vi "Plugin_Collect_Result.vi"(8 "error in (no error)":errorcluster={"status"=FALSE, "code"=0, "source"="\"\""}, 10 "output data":string, 11 "Instance ID":string) -> (0 "error out":errorcluster={"status"=FALSE, "code"=0, "source"="\"\""}, 2 "status ok":bool, 3 "Typed results/event":string)   [LabVIEW 2026]
doc: "INTENT: Validate plugin result payload. LOGIC: Check result type, units, IDs, completion status and attach to current run."
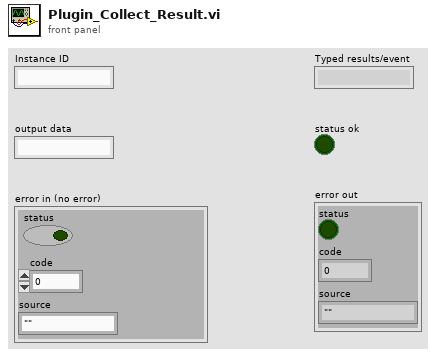
[diagram p1: front panel]
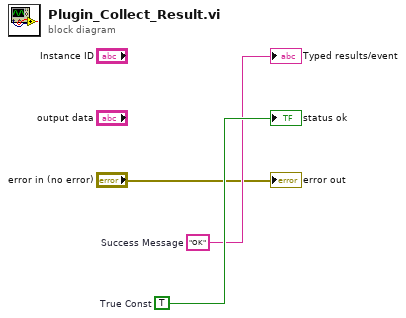
[diagram p0: block diagram]
diagram:
  w3 = TRUE  # True Const
  w2 = "OK"  # Success Message
  "Typed results/event" <- w2
  "status ok" <- w3
  "error out" <- "error in (no error)"
